vi "SUMULADOR VUELO.vi"() -> ()   [LabVIEW 2019]
uses:
  <vilib>/robotics/Controls/Attitude Indicator/Attitude Indicator.xctl
  <vilib>/Instr/_visa.llb/Select Event Type.ctl
  <vilib>/Instr/_visa.llb/VISA Configure Serial Port (Instr).vi
panel:
  in  "VISA resource name":refnum<visa-resource-name>
  in  "stop":bool
  out "Attitude Indicator":cluster{"Roll":dbl, "Pitch":dbl}(xcontrol)
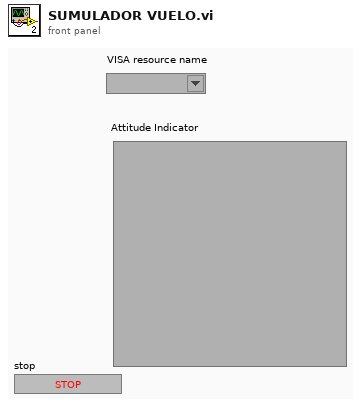
[diagram p1: front panel]
types:
  T1 = typedef "Select Event Type.ctl" = u32
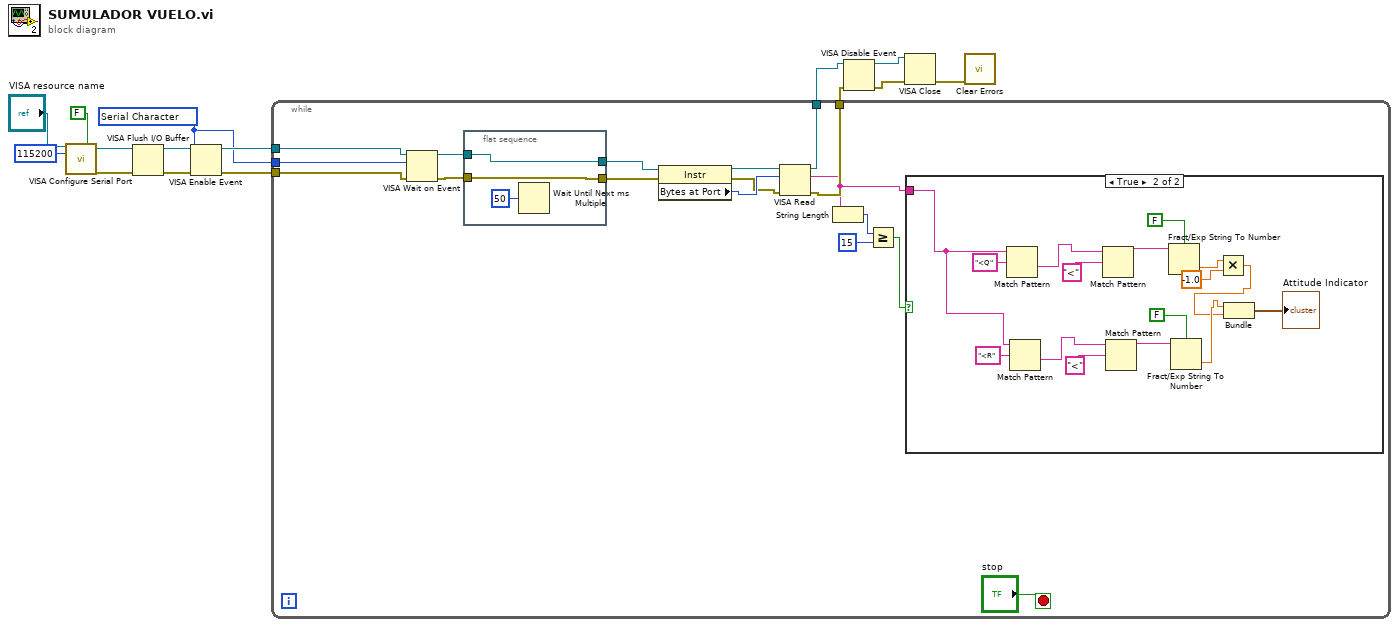
[diagram p0: block diagram]
diagram:
  w6 = T1 1073684533 items=["Service Request"=1073684491, "Trigger"=3221168138, "Clear"=1073684493, "VXI Signal"=1073684512, "VXI/VME Interrupt"=3221168161, "VXI/VME Sysfail"=1073684509, "VXI/VME Sysreset"=1073684510, "GPIB CIC"=1073684498, "GPIB Talk"=1073684499, "GPIB Listen"=1073684500, "PXI Interrupt"=1073684514, "Serial Break"=1073684515, "Serial TermChar"=1073684516, "Serial CTS"=1073684521, "Serial DSR"=1073684522, "Serial DCD"=1073684524, "Serial RI"=1073684526, "Serial Character"=1073684533, "USB Interrupt"=1073684535, "All Enabled"=1073709055] ("Event Type")
  n1 = call-poly "VISA Configure Serial Port"("VISA resource name"="VISA resource name", "Enable Termination\nChar (T)"=FALSE ("Enable Termination\nChar (T)"), "baud rate (9600)"=u32 115200) -> ("VISA resource name out"=w12:refnum<visa-resource-name>, "error out"=w11:errorcluster)  [unwired: 11 in]
  n2 = VISA Flush I/O Buffer(VISA resource name=w12, error in (no error)=w11) -> (VISA resource name out=w10:refnum<visa-resource-name>, error out=w9:errorcluster)  [unwired: 1 in]
  n3 = VISA Enable Event(8:w9, 10:w6, 11:w10) -> (0:w7:errorcluster, 3:w8:refnum<visa-resource-name>)  [unwired: 1 in]
  n4 = while {
    tunnel: w8 -> [w31]
    tunnel: w7 -> [w30]
    tunnel: w6 -> [w29]
    tunnel: [w21] -> w5
    tunnel: [w20] -> w4
    stop <- "stop" stop-if-true
    n5 = VISA Wait on Event(8:w30, 10:w29, 11:w31) -> (0:w26:errorcluster, 3:w27:refnum<visa-resource-name>)  [unwired: 2 in, 2 out]
    n6 = flat-sequence {
      tunnel: [w50] -> w28
      tunnel: w27 -> [w50]
      tunnel: w26 -> [w49]
      tunnel: [w49] -> w25
      frame #0 {
        n7 = Wait Until Next ms Multiple(millisecond multiple=u32 50) -> ()  [unwired: 1 out]
      }
    }
    n8 = property class="Instr"(reference=w28, error in=w25) -> (reference out=w24:refnum<visa-resource-name>, error out=w22:errorcluster, "Bytes at Port"=w23:u32)
    n9 = VISA Read(VISA resource name=w24, byte count=w23, error in (no error)=w22) -> (VISA resource name out=w20:refnum<visa-resource-name>, read buffer=w16:string, error out=w21:errorcluster)  [unwired: 1 out]
    n10 = String Length(string=w16) -> (length=w19:i32)
    n11 = Greater Or Equal?(x=w19, y=15) -> (x >= y?=w17:bool)
    n12 = case shown="True" w17 {
      tunnel: w16 -> [_ w42]
      frame False {
      }
      frame True {
        n13 = Match Pattern(string=w42, regular expression="<Q") -> (after substring=w47:string)  [unwired: 1 in, 3 out]
        n14 = Match Pattern(string=w42, regular expression="<R") -> (after substring=w44:string)  [unwired: 1 in, 3 out]
        n15 = Match Pattern(string=w47, regular expression="<") -> (before substring=w41:string)  [unwired: 1 in, 3 out]
        n16 = Match Pattern(string=w44, regular expression="<") -> (before substring=w39:string)  [unwired: 1 in, 3 out]
        n17 = Fract/Exp String To Number(use system decimal point (T)=FALSE, string=w41) -> (number=w35:dbl)  [unwired: 2 in, 1 out]
        n18 = Fract/Exp String To Number(use system decimal point (T)=FALSE, string=w39) -> (number=w37:dbl)  [unwired: 2 in, 1 out]
        n19 = Multiply(x=w35, y=-1.0) -> (x*y=w33:dbl)
        n20 = Bundle(w37, w33) -> (→"Attitude Indicator":cluster{dbl, dbl})  [unwired: 1 in]
      }
    }
  }
  n21 = VISA Disable Event(8:w5, 11:w4) -> (0:w2:errorcluster, 3:w3:refnum<visa-resource-name>)  [unwired: 2 in]
  n22 = VISA Close(VISA resource name=w3, error in (no error)=w2) -> (error out=w1:errorcluster)
  n23 = call <vilib>:"Clear Errors.vi"("error in (no error)"=w1) -> ()  [unwired: 5 in, 2 out]
